vi "test_DuplicateClientNames_CheckClientNameIsNotRepeated_NameInvalid.vi"() -> (6 "pass":bool, 8 "result":string, 15 "error out":errorcluster)   [LabVIEW 2021, in "MeasurementGenerator Tests.lvlib"]
uses:
  MeasurementGenerator Tests.lvlib
  <vilib>/ErrorRing/Error Ring.xnode
  Generator/_MeasurementClient Utility/MeasurementClient Editor.lvlib
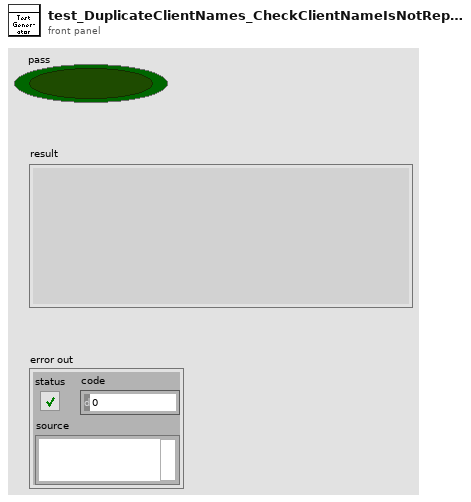
[diagram p1: front panel]
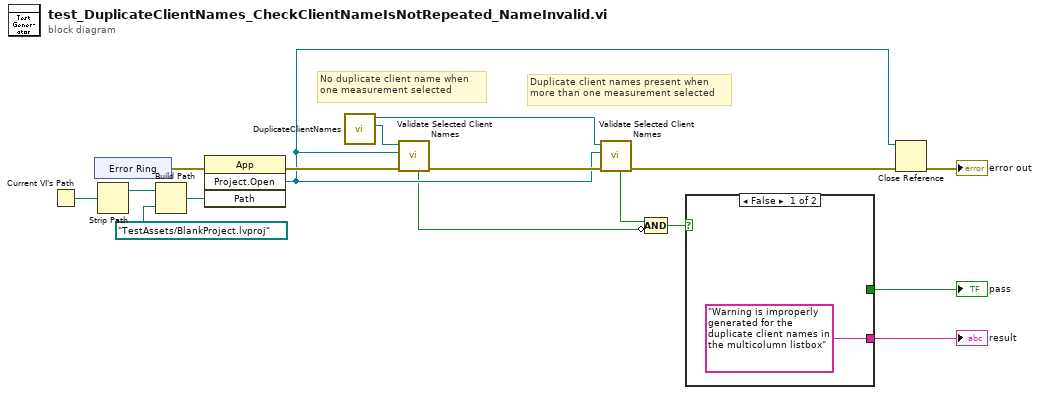
[diagram p0: block diagram]
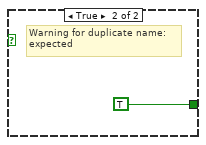
[diagram p2: hidden frame]
diagram:
  # "Duplicate client names present when\nmore than one measurement selected"
  # "No duplicate client name when\none measurement selected"
  n1 = Current VI's Path() -> (path=w17:path)
  n2 = xnode "Error Ring"() -> ("error out"=w14:errorcluster)
  n3 = Strip Path(path=w17) -> (stripped path=w16:path)  [unwired: 1 out]
  n4 = Build Path(base path=w16, name or relative path=path "TestAssets/BlankProject.lvproj" ("path")) -> (appended path=w13:path)
  n5 = invoke class="App" method="Project.Open"(error in=w14, "Path"=w13) -> (error out=w11:errorcluster, "Project:Open"=w4:refnum<vi>)  [unwired: 2 in, 2 out]
  n6 = call "DuplicateClientNames.vi"() -> ("one select refnum"=w7:refnum<vi>, "all select refnum"=w5:refnum<vi>)  [unwired: 10 in]
  n7 = call "Validate Selected Client Names.vi"("error in (no error)"=w11, "project ref"=w4, "multicolumnListbox in"=w7) -> ("error out"=w12:errorcluster, "warning?"=w2:bool)  [unwired: 4 in, 3 out]
  n8 = call "Validate Selected Client Names.vi"("error in (no error)"=w12, "project ref"=w4, "multicolumnListbox in"=w5) -> ("error out"=w6:errorcluster, "warning?"=w3:bool)  [unwired: 4 in, 3 out]
  n9 = Compound Arithmetic op=AND(w3, invert w2) -> (w1:bool)
  n10 = case shown="False" w1 {
    tunnel: ["Warning is improperly generated for the duplicate client names in the multicolumn listbox" ("format string") _] -> w8
    tunnel: [_ TRUE] -> w10
    frame False {
    }
    frame True {
      # "Warning for duplicate name:\nexpected"
    }
  }
  "pass" <- w10
  "result" <- w8
  n11 = Close Reference(reference=w4, error in (no error)=w6) -> (error out=→"error out":errorcluster)
